vi "New Frame Trigger.vi"(8 "error in":errorcluster, 11 "CaptureDetectionLoopDataIn":T1={"Period"=-1, "Reset"=TRUE, "Iteration"=0, "Capture"=path "", "Mode"={"Replay"=enum."None", "Record"=enum."None"}, "Replay Run ID"="", "Frame Number"=0, "Core Module ID"=0, "EventRecorderLaunched"=FALSE, "Frame 0 relative seconds"=0.0, "Record Run ID"=""} {"Frame 0 relative seconds" format="%_19f"}) -> (0 "error out":errorcluster, 1 "Trigger":bool, 2 "Latest Frame":path, 3 "CaptureDetectionLoopDataOut":T1={"Period"=-1, "Reset"=TRUE, "Iteration"=0, "Capture"=path "", "Mode"={"Replay"=enum."None", "Record"=enum."None"}, "Replay Run ID"="", "Frame Number"=0, "Core Module ID"=0, "EventRecorderLaunched"=FALSE, "Frame 0 relative seconds"=0.0, "Record Run ID"=""} {"Frame 0 relative seconds" format="%_19f"})   [LabVIEW 2026, in "Launcher.lvlib"]
uses:
  Launcher.lvlib
  Capture detection loop data--cluster.ctl
  Mode.ctl
  ReplayMode.ctl
  RecordMode.ctl
  Core/global.vi
  Core/Core.lvlib
panel:
  out "Numeric":i32
  out "Number of frames":u32
  out "Throttle":u32
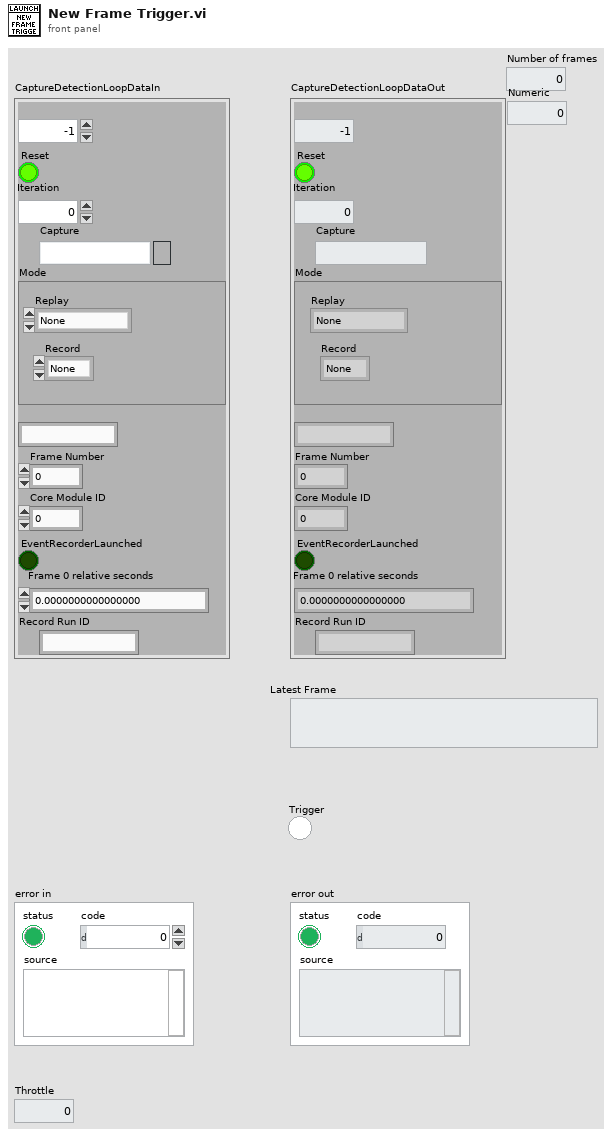
[diagram p1: front panel]
types:
  T1 = typedef "Capture detection loop data--cluster.ctl" = cluster{"Period":i32, "Reset":bool, "Iteration":i32, "Capture":path, "Mode":T2, "Replay Run ID":string, "Frame Number":u32, "Core Module ID":i32, "EventRecorderLaunched":bool, "Frame 0 relative seconds":dbl, "Record Run ID":string}
  T2 = typedef "Mode.ctl" = cluster{"Replay":T3, "Record":T4}
  T3 = typedef "ReplayMode.ctl" = enum16{"None", "User Events"}
  T4 = typedef "RecordMode.ctl" = enum16{"None", "User Events", "Benchmarks", "User Events and Benchmarks"}
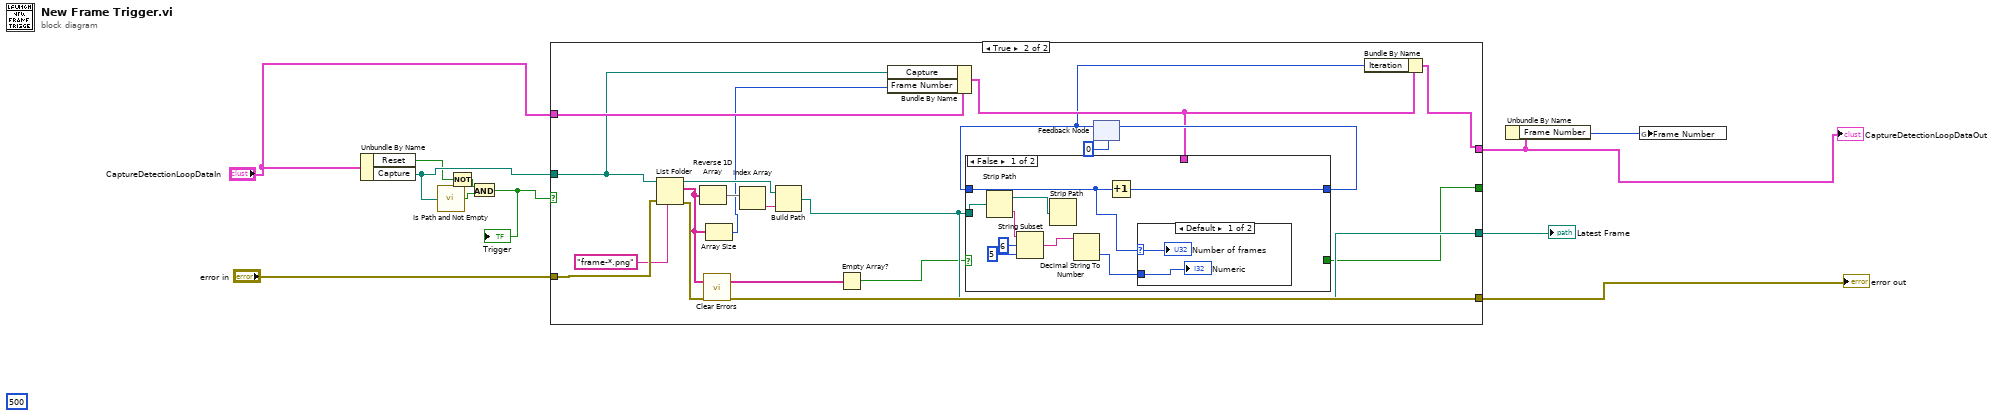
[diagram p0: block diagram]
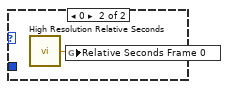
[diagram p3: hidden frame]
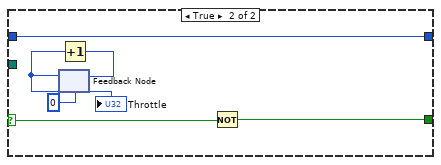
[diagram p4: hidden frame]
diagram:
  (unwired) 500
  n1 = Unbundle By Name("CaptureDetectionLoopDataIn") -> ("Reset"=w3:bool, "Capture"=w6:path)
  n2 = call <vilib>:"Is Path and Not Empty.vi"("path"=w6) -> ("Is Path and Not Empty?"=w9:bool)  [unwired: 4 in]
  n3 = Not(x=w3) -> (.not. x?=w8:bool)
  n4 = And(x=w8, y=w9) -> (x .and. y?=w4:bool)
  "Trigger" <- w4
  n5 = case shown="True" w4 {
    tunnel: "error in" -> [w13 w32]
    tunnel: [w13 w31] -> w10
    tunnel: "CaptureDetectionLoopDataIn" -> [w12 w22]
    tunnel: w6 -> [_ w21]
    tunnel: [_ w23] -> w5
    tunnel: [_ w20] -> _
    tunnel: [w12 w15] -> w2
    frame False {
    }
    frame True {
      n6 = List Folder(path=w21, pattern="frame-*.png", error in=w32) -> (path out=w27:path, filenames=w18:string[], error out=w24:errorcluster)  [unwired: 1 in, 1 out]
      n7 = Reverse 1D Array(array=w18) -> (reversed array=w30:string[])
      n8 = call <vilib>:"Clear Errors.vi"("error in (no error)"=w24) -> ("error out"=w31:errorcluster)  [unwired: 5 in, 1 out]
      n9 = Array Size(array=w18) -> (size(s)=w19:i32)
      n10 = Index Array(array=w30) -> (element=w29:string)  [unwired: 1 in]
      n11 = Build Path(base path=w27, name or relative path=w29) -> (appended path=w23:path)
      n12 = Empty Array?(array=w18) -> (empty?=w17:bool)
      n13 = Bundle By Name(cluster=w22, "Capture"=w21, "Frame Number"=w19) -> (w16:T1)
      n14 = feedback #1(u32 0 ("Number of frames")) -> (w14:u32)
      n15 = case shown="False" w17 {
        selector: w17 -> [_ w46]
        tunnel: w23 -> [w41 _]
        tunnel: [w33 w47] -> w25
        tunnel: w14 -> [w35 w47]
        tunnel: [_ w45] -> w20
        tunnel: w16 -> [_ _]
        frame False {
          n16 = Strip Path(path=w41) -> (stripped path=w40:path, name=w39:string)
          n17 = String Subset(string=w39, offset (0)=6, length (rest)=5 ("length (rest)")) -> (substring=w36:string)
          n18 = Strip Path(path=w40) -> ()  [unwired: 2 out]
          n19 = Decimal String To Number(string=w36) -> (number=w34:i32)  [unwired: 2 in, 1 out]
          n20 = Increment(x=w35) -> (x+1=w33:u32)
          n21 = case shown="Default" w35 {
            selector: w35 -> [w43 _]
            tunnel: w34 -> [w42 _]
            frame Default {
              "Number of frames" <- w43
              "Numeric" <- w42
            }
            frame 0 {
              n22 = call <vilib>:"High Resolution Relative Seconds.vi"() -> ("relative seconds"=w44:dbl)
              n23 = global write "global.vi" "Relative Seconds Frame 0"(w44) -> ()
            }
          }
        }
        frame True {
          n24 = feedback #2(u32 0 ("Number of frames")) -> (w48:u32)
          "Throttle" <- w48
          n25 = Increment(x=w48) -> (x+1=w49:u32)
          n26 = feedback-in #2(w49) -> ()
          n27 = Not(x=w46) -> (.not. x?=w45:bool)
        }
      }
      n28 = feedback-in #1(w25) -> ()
      n29 = Bundle By Name(cluster=w16, "Iteration"=w14) -> (w15:T1)
    }
  }
  "CaptureDetectionLoopDataOut" <- w2
  "error out" <- w10
  "Latest Frame" <- w5
  n30 = Unbundle By Name(w2) -> ("Frame Number"=w1:u32)
  n31 = global write "global.vi" "Frame Number"(w1) -> ()
